vi "Test Get Accounts File Path.vi"() -> ()   [LabVIEW 2026]
doc: "Caraya unit test for Get Accounts File Path.vi. Read-only: the shipped ATM accounts.txt is only checked for existence, never opened.\n\nCase 1: the returned path names the file ATM accounts.txt and that file exists - i.e. the path is built from the VI's own location and points at the accounts file next to the main VI, as the exam requires, in whatever folder the repository is checked out.\n\nThe error cluster carries the FIRST failure only. Read the JUnit report for all of them."
uses:
  <vilib>/addons/_JKI Toolkits/Caraya/classes/Test/Test.lvclass
  <vilib>/addons/_JKI Toolkits/Caraya/classes/Assert/Assert.lvclass
panel:
  out "error out":errorcluster
  in  "error in":errorcluster
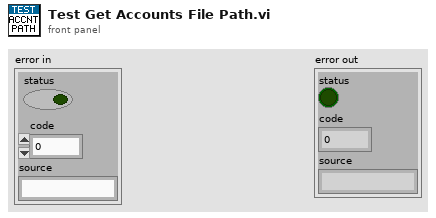
[diagram p1: front panel]
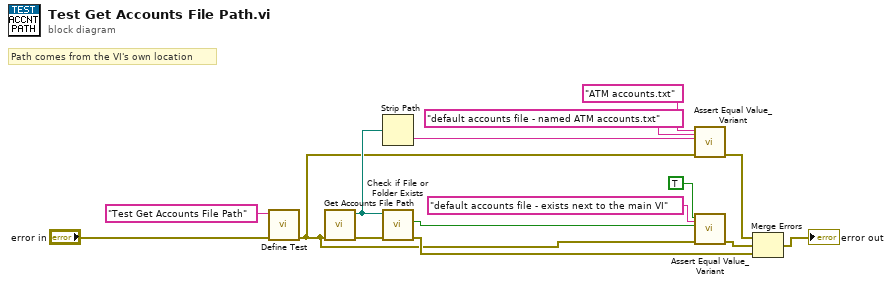
[diagram p0: block diagram]
diagram:
  # "Path comes from the VI's own location"
  n1 = call <vilib>:"Define Test.vi"("error in (no error)"="error in", "Label (VI Title)"="Test Get Accounts File Path") -> ("error out"=w4:errorcluster)  [unwired: 8 in, 1 out]
  n2 = call "Get Accounts File Path.vi"("error in"=w4) -> ("error out"=w6:errorcluster, "Accounts File Path"=w5:path)  [unwired: 9 in]
  n3 = Strip Path(path=w5) -> (name=w7:string)  [unwired: 1 out]
  n4 = call <vilib>:"Check if File or Folder Exists.vi"("error in (no error)"=w6, "path"=w5) -> ("error out"=w8:errorcluster, "file or folder exists?"=w9:bool)  [unwired: 7 in, 1 out]
  n5 = call <vilib>:"Assert Equal Value_Variant.vi"("Label"="default accounts file - named ATM accounts.txt", "error in (no error)"=w4, "Actual"=w7, "Expected"="ATM accounts.txt" ("expected 1")) -> ("error out"=w12:errorcluster)  [unwired: 6 in, 1 out]
  n6 = call <vilib>:"Assert Equal Value_Variant.vi"("Label"="default accounts file - exists next to the main VI", "error in (no error)"=w4, "Actual"=w9, "Expected"=TRUE ("expected 2")) -> ("error out"=w15:errorcluster)  [unwired: 6 in, 1 out]
  n7 = Merge Errors(w12, w15, w8) -> (→"error out":errorcluster)
